vi "Get Server Certificates (Client).vi"(10 "Server Certificates":T1) -> (2 "trusted server certificates":path[](array[path]))   [LabVIEW 2014, in "OPC UA Client runtime.lvclass"]
doc: "Get paths to trusted server certificates used in creating an OPC UA Client connection"
uses:
  OPC UA Client runtime.lvclass
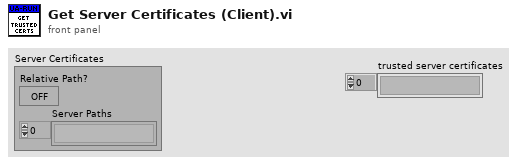
[diagram p1: front panel]
types:
  T1 = cluster{"Relative Path?":bool, "Server Paths":string[]}
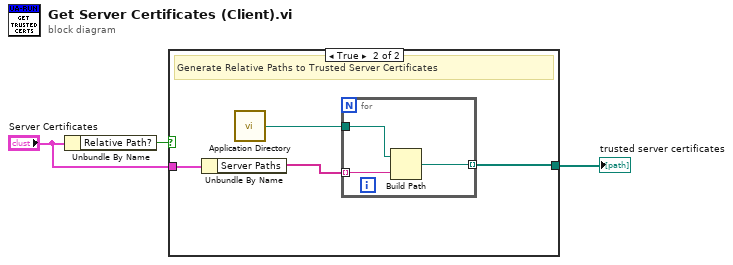
[diagram p0: block diagram]
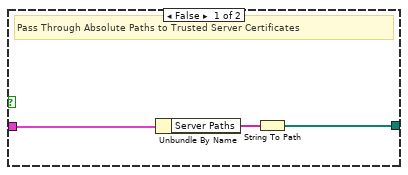
[diagram p2: hidden frame]
diagram:
  n1 = Unbundle By Name("Server Certificates") -> ("Relative Path?"=w3:bool)
  n2 = case shown="True" w3 {
    tunnel: "Server Certificates" -> [w6 w10]
    tunnel: [w4 w8] -> w1
    frame False {
      # "Pass Through Absolute Paths to Trusted Server Certificates"
      n3 = Unbundle By Name(w6) -> ("Server Paths"=w5:string[])
      n4 = String To Path(string=w5) -> (path=w4:path[])
    }
    frame True {
      # "Generate Relative Paths to Trusted Server Certificates"
      n5 = Unbundle By Name(w10) -> ("Server Paths"=w9:string[])
      n6 = call <vilib>:"Application Directory.vi"() -> ("Application Directory"=w7:path)
      n7 = for {
        tunnel: w9 -> [w13] mode=indexing
        tunnel: [w12] -> w8 mode=indexing
        tunnel: w7 -> [w11]
        n8 = Build Path(base path=w11, name or relative path=w13) -> (appended path=w12:path)
      }
    }
  }
  "trusted server certificates" <- w1
